vi "Get View.vi"(8 "error in":errorcluster, 11 "Cell in":refnum<class "Cell.lvclass">) -> (0 "error out":errorcluster, 2 "View":refnum<class "Cell View.lvclass">, 3 "Cell out":refnum<class "Cell.lvclass">)   [LabVIEW 2020, in "SourceGrid.lvlib" / "Cell.lvclass"]
uses:
  Cell.lvclass
  Views/Cell View/Cell View.lvclass
  Cell.lvclass/Cell.ctl
  D:/git/Sourcegrid-LabVIEW/source/SourceGrid.dll
  SourceGrid.dll
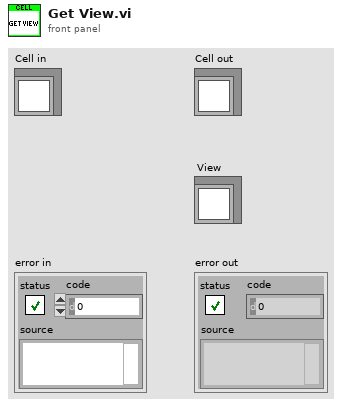
[diagram p1: front panel]
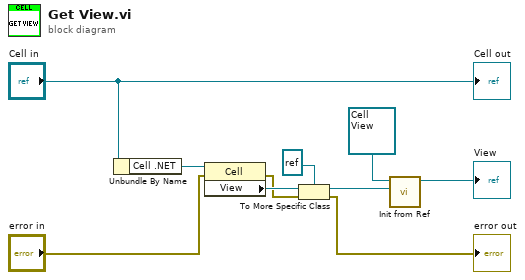
[diagram p0: block diagram]
diagram:
  n1 = Unbundle By Name("Cell in") -> ("Cell .NET"=w9:refnum<k24>)
  n2 = property class="Cell"(reference=w9, error in="error in") -> (error out=w4:errorcluster, "View"=w7:refnum<k24>)  [unwired: 1 out]
  n3 = To More Specific Class(target class=refnum<k24> refnum ("new reference"), reference=w7, error in=w4) -> (specific class reference=w1:refnum<k24>, error out=→"error out":errorcluster)
  n4 = call-dynamic "Init from Ref.vi"("Cell View .NET"=w1, "Cell View in"=refnum<class "Cell View.lvclass"> refnum) -> ("Cell View out"=→"View":refnum<class "Cell View.lvclass">)  [unwired: 9 in]
  "Cell out" <- "Cell in"
